vi "USBPT104Example.vi"() -> ()   [LabVIEW 2010]
panel:
  in  "Channel Filters":i16(ring) items=["Off", "On"]
  in  "SetMains":u16(ring) items=["50 Hz", "60 Hz"]
  out "Ch4 Status":enum32{"Red", "Yellow", "Green"}(radio)
  out "Ch3 Status":enum32{"Red", "Yellow", "Green"}(radio)
  out "GetValue PICO_STATUS log":T1(array[cluster]) {"Hex Code" format="%x"}
  out "Ch2 Status":enum32{"Red", "Yellow", "Green"}(radio)
  out "Ch1 Status":enum32{"Red", "Yellow", "Green"}(radio)
  out "CH4 Value":dbl(slide)=nan min=-200.0 max=800.0 scale=0.0..115.0
  out "CH3 Value":dbl(slide)=nan min=-200.0 max=800.0 scale=0.0..10000.0
  out "CH2 Value":dbl(slide)=nan min=-200.0 max=800.0 scale=-200.0..800.0
  out "CH1 Value":dbl(slide)=nan min=0.0 max=375.0 scale=-200.0..800.0
  in  "Channel Settings":T2={"CH1 # Wires"=4, "CH1 Measurement Type"=1, "CH2 # Wires"=2, "CH2 Measurement Type"=0, "CH3 # Wires"=2, "CH3 Measurement Type"=0, "CH4 # Wires"=2, "CH4 Measurement Type"=0} {"CH4 Measurement Type" items=["OFF", "PT100", "PT1000", "Resistance to 375 Ohms", "Resistance to 10 kOhms"]; "CH4 # Wires" items=["2"=2, "3"=3, "4"=4]; "CH3 Measurement Type" items=["OFF", "PT100", "PT1000", "Resistance to 375 Ohms", "Resistance to 10 kOhms"]; "CH3 # Wires" items=["2"=2, "3"=3, "4"=4]; "CH2 Measurement Type" items=["OFF", "PT100", "PT1000", "Resistance to 375 Ohms", "Resistance to 10 kOhms"]; "CH2 # Wires" items=["2"=2, "3"=3, "4"=4]; "CH1 Measurement Type" items=["OFF", "PT100", "PT1000", "Resistance to 375 Ohms", "Resistance to 10 kOhms"]; "CH1 # Wires" items=["2"=2, "3"=3, "4"=4]}
  out "Unit Info":T3
  in  "Connection":bool=TRUE
  in  "Use Serial Number":bool
  in  "Serial Number":string
  in  "IP Address:port number":string="192.168.1.30:6250"
  out "PT-104 Units":string
  in  "error in (no error)":errorcluster
  out "End time":timestamp=timestamp(-9593251199.456087 s since 1904-01-01)
  out "Start time":timestamp=timestamp(-9593251199.456087 s since 1904-01-01)
  out "error out":errorcluster
  in  "Update settings":bool
  in  "Stop":bool
  # "USB"
  # "Ethernet"
  # "Channel Status LED-\nYellow- Waiting/Off\nGreen- Read OK\nRed- Read Error"
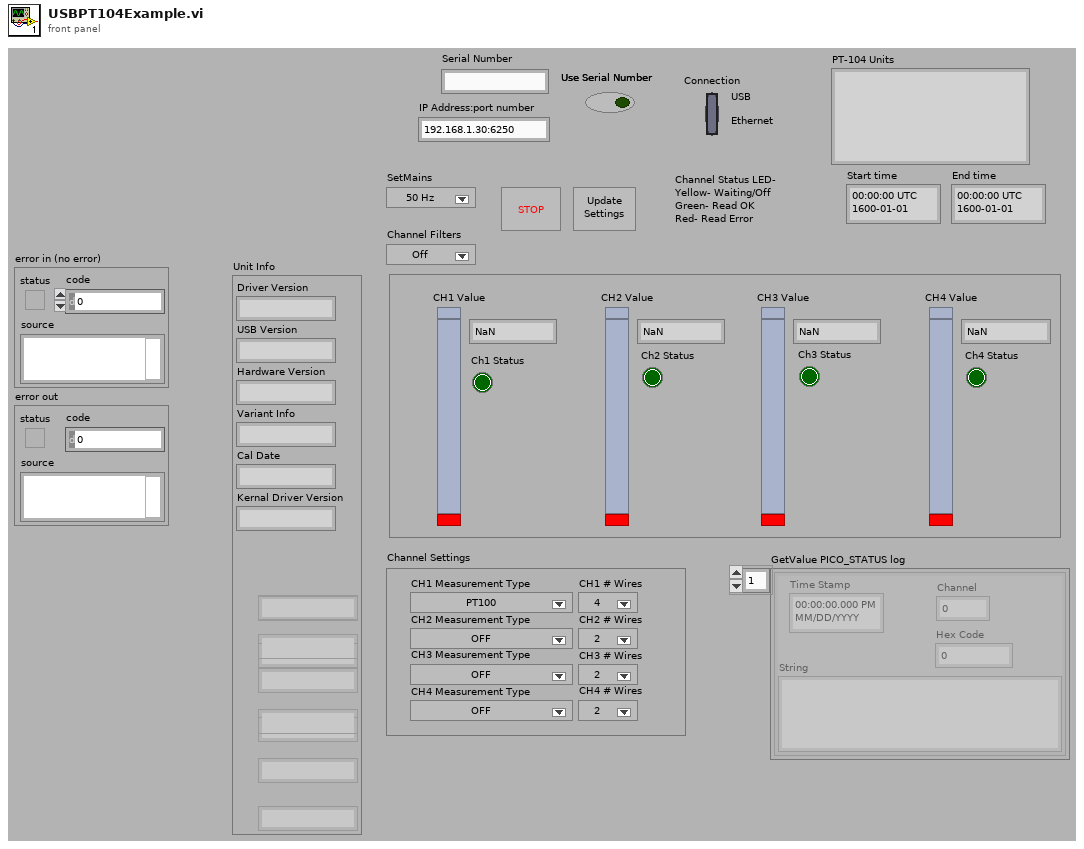
[diagram p1: front panel]
types:
  T1 = cluster{"Time Stamp":timestamp, "Hex Code":i32, "String":string, "Channel":i32}[]
  T2 = cluster{"CH1 # Wires":i16, "CH1 Measurement Type":i32, "CH2 # Wires":i16, "CH2 Measurement Type":i32, "CH3 # Wires":i16, "CH3 Measurement Type":i32, "CH4 # Wires":i16, "CH4 Measurement Type":i32}
  T3 = cluster{"Driver Version":string, "USB Version":string, "Hardware Version":string, "Variant Info":string, "Cal Date":string, "Kernal Driver Version":string, "NA":string, "NA 2":string, "NA":string, "NA 3":string, "NA 4":string, "NA 5":string, "NA 6":string, "NA 7":string, "NA 8":string}
  T4 = cluster{"seconds since 1Jan1904":timestamp, u32, "String":string, i32}[]
  T5 = cluster{"status":bool, "code":u32, "source":string}
  T6 = cluster{"Channel Value":dbl, "Data Range:Maximum":dbl, "Scale.Range:Minimum":dbl}
  T7 = cluster{"seconds since 1Jan1904":timestamp, "code":u32, "String":string, i32}
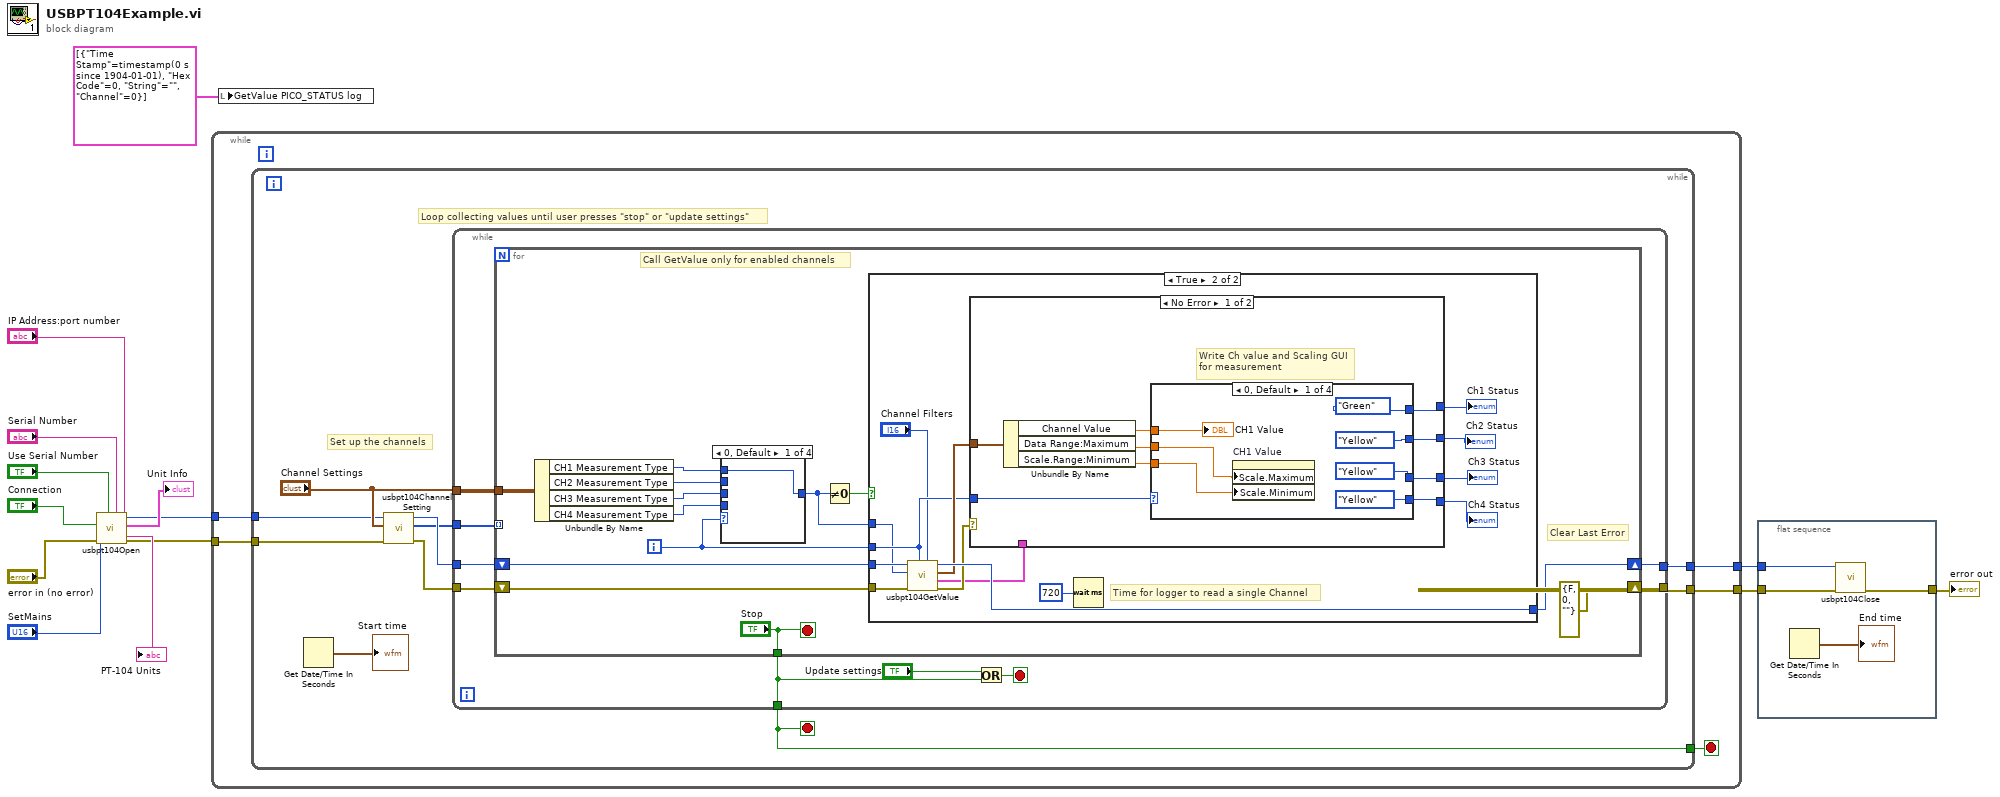
[diagram p0: block diagram]
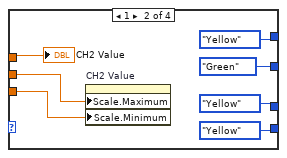
[diagram p6: hidden frame]
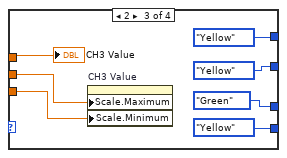
[diagram p7: hidden frame]
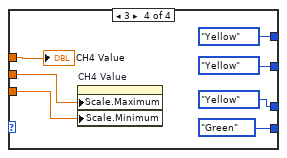
[diagram p8: hidden frame]
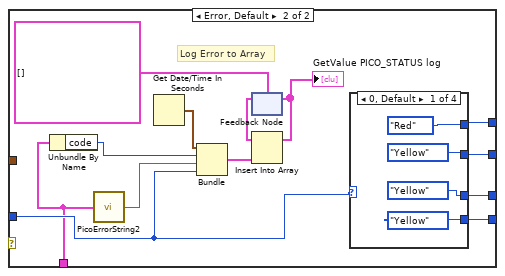
[diagram p9: hidden frame]
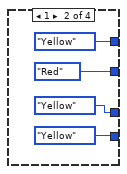
[diagram p10: hidden frame]
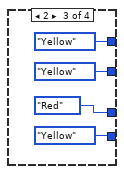
[diagram p11: hidden frame]
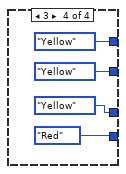
[diagram p12: hidden frame]
diagram:
  n1 = call "usbpt104Open.vi"("IP Address:port number"="IP Address:port number", "Serial Number"="Serial Number", "Use Serial Number"="Use Serial Number", "error in (no error)"="error in (no error)", "Connection"="Connection", "SetMains"="SetMains") -> ("error out"=w7:errorcluster, "Unit Info"=→"Unit Info":T3, "handle out"=w6:i16, "PT-104 Units"=→"PT-104 Units":string)  [unwired: 1 in, 1 out]
  n2 = while {
    tunnel: w7 -> [w19]
    tunnel: w6 -> [w18]
    tunnel: [w16] -> w5
    tunnel: [w15] -> w4
    stop <- w17 stop-if-true
    n3 = while {
      tunnel: [w29] -> w16
      tunnel: [w28] -> w15
      tunnel: [w24] -> w17
      tunnel: w19 -> [w23]
      tunnel: w18 -> [w22]
      stop <- w24 stop-if-true
      # "Loop collecting values until user presses \"stop\" or \"update settings\""
      # "Set up the channels"
      n4 = Get Date/Time In Seconds() -> (seconds since 1Jan1904=→"Start time":timestamp)
      n5 = call "usbpt104ChannelSetting.vi"("error in (no error)"=w23, "Channel Settings"="Channel Settings", "Handle In"=w22) -> ("error out"=w27:errorcluster, "Channel Enable Array"=w20:u8[], "Handle out"=w26:i16)  [unwired: 6 in]
      n6 = while {
        tunnel: w26 -> [w38]
        tunnel: w27 -> [w37]
        tunnel: [w34] -> w29
        tunnel: [w33] -> w28
        tunnel: [w31] -> w24
        tunnel: "Channel Settings" -> [w32]
        tunnel: w20 -> [w30]
        stop <- w36 stop-if-true
        n7 = for {
          shift-right: [errorcluster {"status"=FALSE, "code"=0, "source"=""} ("error out")] -> w34
          shift-left: w37 -> [w50]
          shift-right: [w48] -> w33
          shift-left: w38 -> [w51]
          tunnel: w32 -> [w46]
          tunnel: ["Stop"] -> w31
          tunnel: w30 -> [_] mode=indexing
          i -> [w47]
          stop <- "Stop" stop-if-true
          # "Clear Last Error"
          # "Call GetValue only for enabled channels"
          n8 = Unbundle By Name(w46) -> ("CH1 Measurement Type"=w45:i32, "CH2 Measurement Type"=w44:i32, "CH3 Measurement Type"=w43:i32, "CH4 Measurement Type"=w42:i32)
          n9 = case shown="0, Default" w47 {
            tunnel: [w52 w53 w54 w55] -> w39
            tunnel: w45 -> [w52 _ _ _]
            tunnel: w44 -> [_ w53 _ _]
            tunnel: w43 -> [_ _ w54 _]
            tunnel: w42 -> [_ _ _ w55]
            frame 0, Default {
            }
            frame 1 {
            }
            frame 2 {
            }
            frame 3 {
            }
          }
          n10 = Not Equal To 0?(x=w39) -> (x != 0?=w49:bool)
          n11 = case shown="True" w49 {
            tunnel: w51 -> [w56 w69]
            tunnel: w50 -> [_ w70]
            tunnel: [w56 w68] -> w48
            tunnel: w47 -> [_ w65]
            tunnel: w39 -> [_ w59]
            frame False {
            }
            frame True {
              # "Time for logger to read a single Channel"
              n12 = call "usbpt104GetValue.vi"("Filter"="Channel Filters", "Channel"=w65, "error in (no error)"=w70, "Measurement Type"=w59, "handle in"=w69) -> ("error out"=w58:errorcluster, "PICO_STATUS out"=w57:T5, "Channel Data"=w66:T6, "handle out"=w68:i16)  [unwired: 3 in]
              n13 = case shown="No Error" w58 {
                tunnel: w66 -> [w79 _]
                tunnel: w65 -> [w78 w113]
                tunnel: [w74 w115] -> w64
                tunnel: [w73 w114] -> w63
                tunnel: [w71 w112] -> w62
                tunnel: [w72 w111] -> w61
                tunnel: w57 -> [_ w109]
                frame No Error {
                  # "Write Ch value and Scaling GUI for measurement"
                  n14 = Unbundle By Name(w79) -> ("Channel Value"=w77:dbl, "Data Range:Maximum"=w76:dbl, "Scale.Range:Minimum"=w75:dbl)
                  n15 = case shown="0, Default" w78 {
                    tunnel: w77 -> [w86 w93 w100 w107]
                    tunnel: w76 -> [w80 w87 w95 w102]
                    tunnel: w75 -> [w81 w88 w94 w101]
                    tunnel: [enum32{"Red", "Yellow", "Green"}."Green" ("Select") enum32{"Red", "Yellow", "Green"}."Yellow" ("Select") enum32{"Red", "Yellow", "Green"}."Yellow" ("Select") enum32{"Red", "Yellow", "Green"}."Yellow" ("Select")] -> w74
                    tunnel: [enum32{"Red", "Yellow", "Green"}."Yellow" ("Select") enum32{"Red", "Yellow", "Green"}."Green" ("Select") enum32{"Red", "Yellow", "Green"}."Yellow" ("Select") enum32{"Red", "Yellow", "Green"}."Yellow" ("Select")] -> w73
                    tunnel: [enum32{"Red", "Yellow", "Green"}."Yellow" ("Select") enum32{"Red", "Yellow", "Green"}."Yellow" ("Select") enum32{"Red", "Yellow", "Green"}."Yellow" ("Select") enum32{"Red", "Yellow", "Green"}."Green" ("Select")] -> w72
                    tunnel: [enum32{"Red", "Yellow", "Green"}."Yellow" ("Select") enum32{"Red", "Yellow", "Green"}."Yellow" ("Select") enum32{"Red", "Yellow", "Green"}."Green" ("Select") enum32{"Red", "Yellow", "Green"}."Yellow" ("Select")] -> w71
                    frame 0, Default {
                      n16 = property on="CH1 Value" class="Slide (strict)"("Scale.Maximum"=w80, "Scale.Minimum"=w81) -> ()  [unwired: 2 in, 2 out]
                      "CH1 Value" <- w86
                    }
                    frame 1 {
                      n17 = property on="CH2 Value" class="Slide (strict)"("Scale.Maximum"=w87, "Scale.Minimum"=w88) -> ()  [unwired: 2 in, 2 out]
                      "CH2 Value" <- w93
                    }
                    frame 2 {
                      n18 = property on="CH3 Value" class="Slide (strict)"("Scale.Maximum"=w95, "Scale.Minimum"=w94) -> ()  [unwired: 2 in, 2 out]
                      "CH3 Value" <- w100
                    }
                    frame 3 {
                      n19 = property on="CH4 Value" class="Slide (strict)"("Scale.Maximum"=w102, "Scale.Minimum"=w101) -> ()  [unwired: 2 in, 2 out]
                      "CH4 Value" <- w107
                    }
                  }
                }
                frame Error, Default {
                  # "Log Error to Array"
                  n20 = Unbundle By Name(w109) -> ("code"=w108:u32)
                  n21 = call "PicoErrorString2.vi"("PICO_STATUS in"=w109) -> ("String"=w116:string)  [unwired: 2 in, 2 out]
                  n22 = Get Date/Time In Seconds() -> (seconds since 1Jan1904=w117:timestamp)
                  n23 = Bundle("seconds since 1Jan1904"=w117, "code"=w108, "String"=w116, w113) -> (w120:T7)  [unwired: 1 in]
                  n24 = feedback #1(T4 []) -> (w118:T4)
                  n25 = Insert Into Array(array=w118, new element=w120) -> (w119:T4)  [unwired: 1 in]
                  "GetValue PICO_STATUS log" <- w119
                  n26 = feedback-in #1(w119) -> ()
                  n27 = case shown="0, Default" w113 {
                    tunnel: [enum32{"Red", "Yellow", "Green"}."Red" ("Select") enum32{"Red", "Yellow", "Green"}."Yellow" ("Select") enum32{"Red", "Yellow", "Green"}."Yellow" ("Select") enum32{"Red", "Yellow", "Green"}."Yellow" ("Select")] -> w115
                    tunnel: [enum32{"Red", "Yellow", "Green"}."Yellow" ("Select") enum32{"Red", "Yellow", "Green"}."Red" ("Select") enum32{"Red", "Yellow", "Green"}."Yellow" ("Select") enum32{"Red", "Yellow", "Green"}."Yellow" ("Select")] -> w114
                    tunnel: [enum32{"Red", "Yellow", "Green"}."Yellow" ("Select") enum32{"Red", "Yellow", "Green"}."Yellow" ("Select") enum32{"Red", "Yellow", "Green"}."Red" ("Select") enum32{"Red", "Yellow", "Green"}."Yellow" ("Select")] -> w112
                    tunnel: [enum32{"Red", "Yellow", "Green"}."Yellow" ("Select") enum32{"Red", "Yellow", "Green"}."Yellow" ("Select") enum32{"Red", "Yellow", "Green"}."Yellow" ("Select") enum32{"Red", "Yellow", "Green"}."Red" ("Select")] -> w111
                    frame 0, Default {
                    }
                    frame 1 {
                    }
                    frame 2 {
                    }
                    frame 3 {
                    }
                  }
                }
              }
              "Ch1 Status" <- w64
              "Ch2 Status" <- w63
              "Ch3 Status" <- w62
              "Ch4 Status" <- w61
              n28 = Wait (ms)(milliseconds to wait=u32 720) -> ()  [unwired: 1 out]
            }
          }
        }
        n29 = Or(x="Update settings", y=w31) -> (x .or. y?=w36:bool)
      }
    }
  }
  n30 = local write "GetValue PICO_STATUS log"(T1 [{"Time Stamp"=timestamp(0 s since 1904-01-01), "Hex Code"=0, "String"="", "Channel"=0}] ("GetValue PICO_STATUS log")) -> ()
  n31 = flat-sequence {
    tunnel: w5 -> [w140]
    tunnel: [w138] -> w3
    tunnel: w4 -> [w139]
    frame #0 {
      n32 = Get Date/Time In Seconds() -> (seconds since 1Jan1904=→"End time":timestamp)
      n33 = call "usbpt104Close.vi"("error in (no error)"=w140, "handle in"=w139) -> ("error out"=w138:errorcluster)  [unwired: 8 in, 1 out]
    }
  }
  "error out" <- w3
